vi "FX232_485_BTWT.vi"(5 "延时":u8 max=150 step=10, 7 "PLC站号":u8=1, 8 "error in (no error)":errorcluster caption="错误输入（无错误）", 9 "地址值":cluster{"地址":string, "值":string}[](array[cluster]), 10 "命令":string(combo)="BT", 11 "Port":refnum<visa-resource-name>) -> (0 "error out":errorcluster caption="错误输出", 1 "成功":bool, 2 "Buff":string, 3 "PortOut":refnum<visa-resource-name>)   [LabVIEW 2025]
uses:
  <vilib>/Utility/error.llb/Trim Whitespace One-Sided.vi
panel:
  out "连接的字符串":string
  # "Y,D,M"
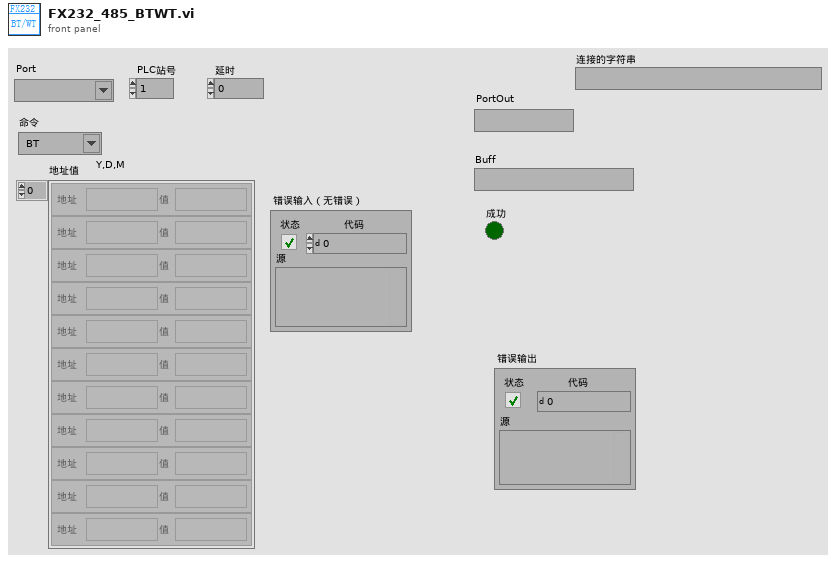
[diagram p1: front panel]
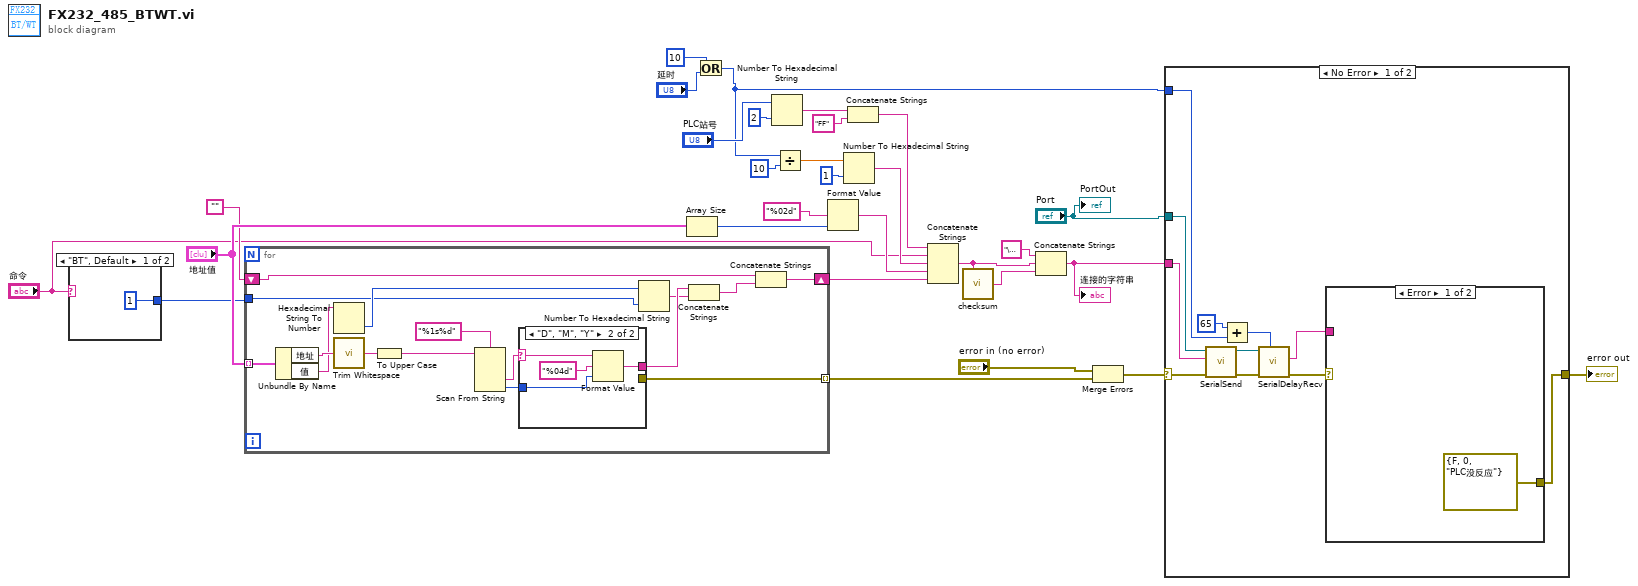
[diagram p0: block diagram]
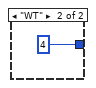
[diagram p2: hidden frame]
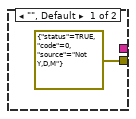
[diagram p3: hidden frame]
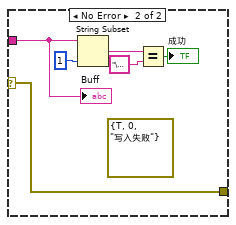
[diagram p4: hidden frame]
diagram:
  n1 = case shown="\"BT\", Default" "命令" {
    tunnel: [1 4] -> w5
    frame "BT", Default {
    }
    frame "WT" {
    }
  }
  n2 = for {
    tunnel: w5 -> [w32]
    tunnel: "地址值" -> [w47] mode=indexing
    tunnel: [w39] -> w14 mode=indexing
    shift-right: [w34] -> w11
    shift-left: "" -> [w35]
    n3 = Unbundle By Name(w47) -> ("地址"=w41:string, "值"=w40:string)
    n4 = Hexadecimal String To Number(string=w40) -> (number=w33:u32)  [unwired: 2 in, 1 out]
    n5 = call <vilib>:"Trim Whitespace.vi"("string"=w41) -> ("trimmed string"=w45:string)  [unwired: 1 in]
    n6 = To Upper Case(1:w45) -> (0:w44:string)
    n7 = Scan From String(format string="%1s%d" ("格式字符串"), input string=w44) -> (output 1=w43:string, output 2=w46:i32)  [unwired: 4 in, 3 out]
    n8 = case shown="\"D\", \"M\", \"Y\"" w43 {
      selector: w43 -> [_ w52]
      tunnel: w46 -> [_ w51]
      tunnel: [errorcluster {"status"=TRUE, "code"=0, "source"="Not Y,D,M"} ("error in (no error)") _] -> w39
      tunnel: [_ w50] -> w38
      frame "", Default {
      }
      frame "D", "M", "Y" {
        n9 = Format Value(string ("")=w52, format string="%04d" ("格式字符串"), value (0)=w51) -> (output string=w50:string)
      }
    }
    n10 = Number To Hexadecimal String(1:w32, 2:w33) -> (0:w37:string)
    n11 = Concatenate Strings(w38, w37) -> (w36:string)
    n12 = Concatenate Strings(w35, w36) -> (w34:string)
  }
  n13 = Array Size(array="地址值") -> (size(s)=w17:i32)
  n14 = Or(x=u8 10, y="延时") -> (x .or. y?=w2:u8)
  n15 = Number To Hexadecimal String(1:i16 2 ("宽度(-)"), 2:"PLC站号") -> (0:w21:string)
  n16 = Divide(x=w2, y=10) -> (x/y=w25:dbl)
  n17 = Format Value(format string="%02d" ("格式字符串"), value (0)=w17) -> (output string=w15:string)  [unwired: 1 in]
  n18 = Number To Hexadecimal String(1:i16 1 ("宽度(-)"), 2:w25) -> (0:w20:string)
  n19 = Concatenate Strings(w21, "FF" ("字符串")) -> (w18:string)
  n20 = Concatenate Strings(w18, "命令", w20, w15, w11) -> (w8:string)
  n21 = call "checksum.vi"("buff"=w8) -> ("checksum"=w7:string)  [unwired: 4 in]
  n22 = Concatenate Strings("\u0005" ("字符串"), w8, w7) -> (w23:string)
  "连接的字符串" <- w23
  n23 = Merge Errors("error in (no error)", w14) -> (w13:errorcluster)
  n24 = case shown="No Error" w13 {
    selector: w13 -> [w61 w71]
    tunnel: w23 -> [w63 _]
    tunnel: "Port" -> [w62 _]
    tunnel: [w60 w71] -> w29
    tunnel: w2 -> [w59 _]
    frame No Error {
      n25 = call "SerialSend.vi"("error in (no error)"=w61, "SendData"=w63, "PORT"=w62) -> ("error out"=w55:errorcluster, "PORT out"=w56:refnum<visa-resource-name>)  [unwired: 6 in, 1 out]
      n26 = Add(x=u32 65 ("等待时间（毫秒）"), y=w59) -> (x+y=w57:u32)
      n27 = call "SerialDelayRecv.vi"("Timeout"=w57, "error in (no error)"=w55, "Port"=w56) -> ("error out"=w53:errorcluster, "Buff"=w54:string)  [unwired: 6 in, 1 out]
      n28 = case shown="Error" w53 {
        selector: w53 -> [_ w65]
        tunnel: [errorcluster {"status"=FALSE, "code"=0, "source"="PLC没反应"} ("错误常量") w65] -> w60
        tunnel: w54 -> [_ w67]
        frame Error {
        }
        frame No Error {
          (unwired) errorcluster {"status"=TRUE, "code"=0, "source"="写入失败"} ("f")
          n29 = String Subset(string=w67, length (rest)=1 ("长度（剩余）")) -> (substring=w69:string)  [unwired: 1 in]
          n30 = Equal?(x=w69, y="\u0006") -> (x = y?=→"成功":bool)
          "Buff" <- w67
        }
      }
    }
    frame Error {
    }
  }
  "error out" <- w29
  "PortOut" <- "Port"
